vi "Append Image to Report (path).vi"(0 "report in":refnum<class "ooWriter.lvclass">, 1 "alignment (default)":T1, 2 "MS Office parameters":T2, 7 "path or URL of image":path, 9 "caption or alternative string":string, 11 "error in (no error)":errorcluster) -> (4 "report out":refnum<class "ooWriter.lvclass">, 8 "start out (Word)":i32, 10 "end out (Word)":i32, 15 "error out":errorcluster)   [LabVIEW 2009, in "ooWriter.lvclass"]
doc: "For an HTML report, the VI embeds a link to an image into the report. For a standard report, the VI appends the image from a file. You can wire either a path to the image or a string that contains the image URL to this polymorphic VI. The data type you wire to the <B>path or URL of image</B> input determines the polymorphic instance to use."
uses:
  ooWriter.lvclass
  <vilib>/Utility/NIReport.llb/HTML Report Image Alignment.ctl
  C:/Projets/LAVAG/OpenOfficeRGT/AODL/DLLs/AODL.dll
  <vilib>/Utility/NIReport.llb/NI_ReportGenerationCore.lvlib
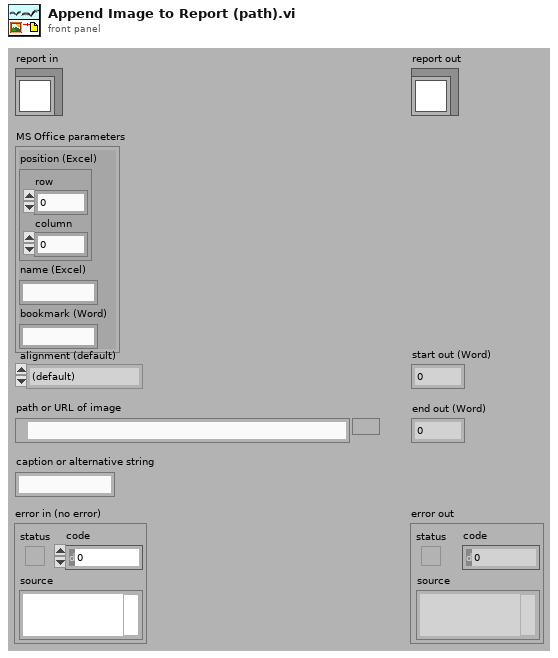
[diagram p1: front panel]
types:
  T1 = typedef "NI_ReportGenerationCore.lvlib/HTML Report Image Alignment.ctl" = enum16{"(default)", "LEFT", "RIGHT", "TOP", "TEXTTOP", "MIDDLE", "ABSMIDDLE", "BASELINE", "BOTTOM", "ABSBOTTOM"}
  T2 = cluster{"position (Excel)":cluster{"row":i32, "column":i32}, "name (Excel)":string, "bookmark (Word)":string}
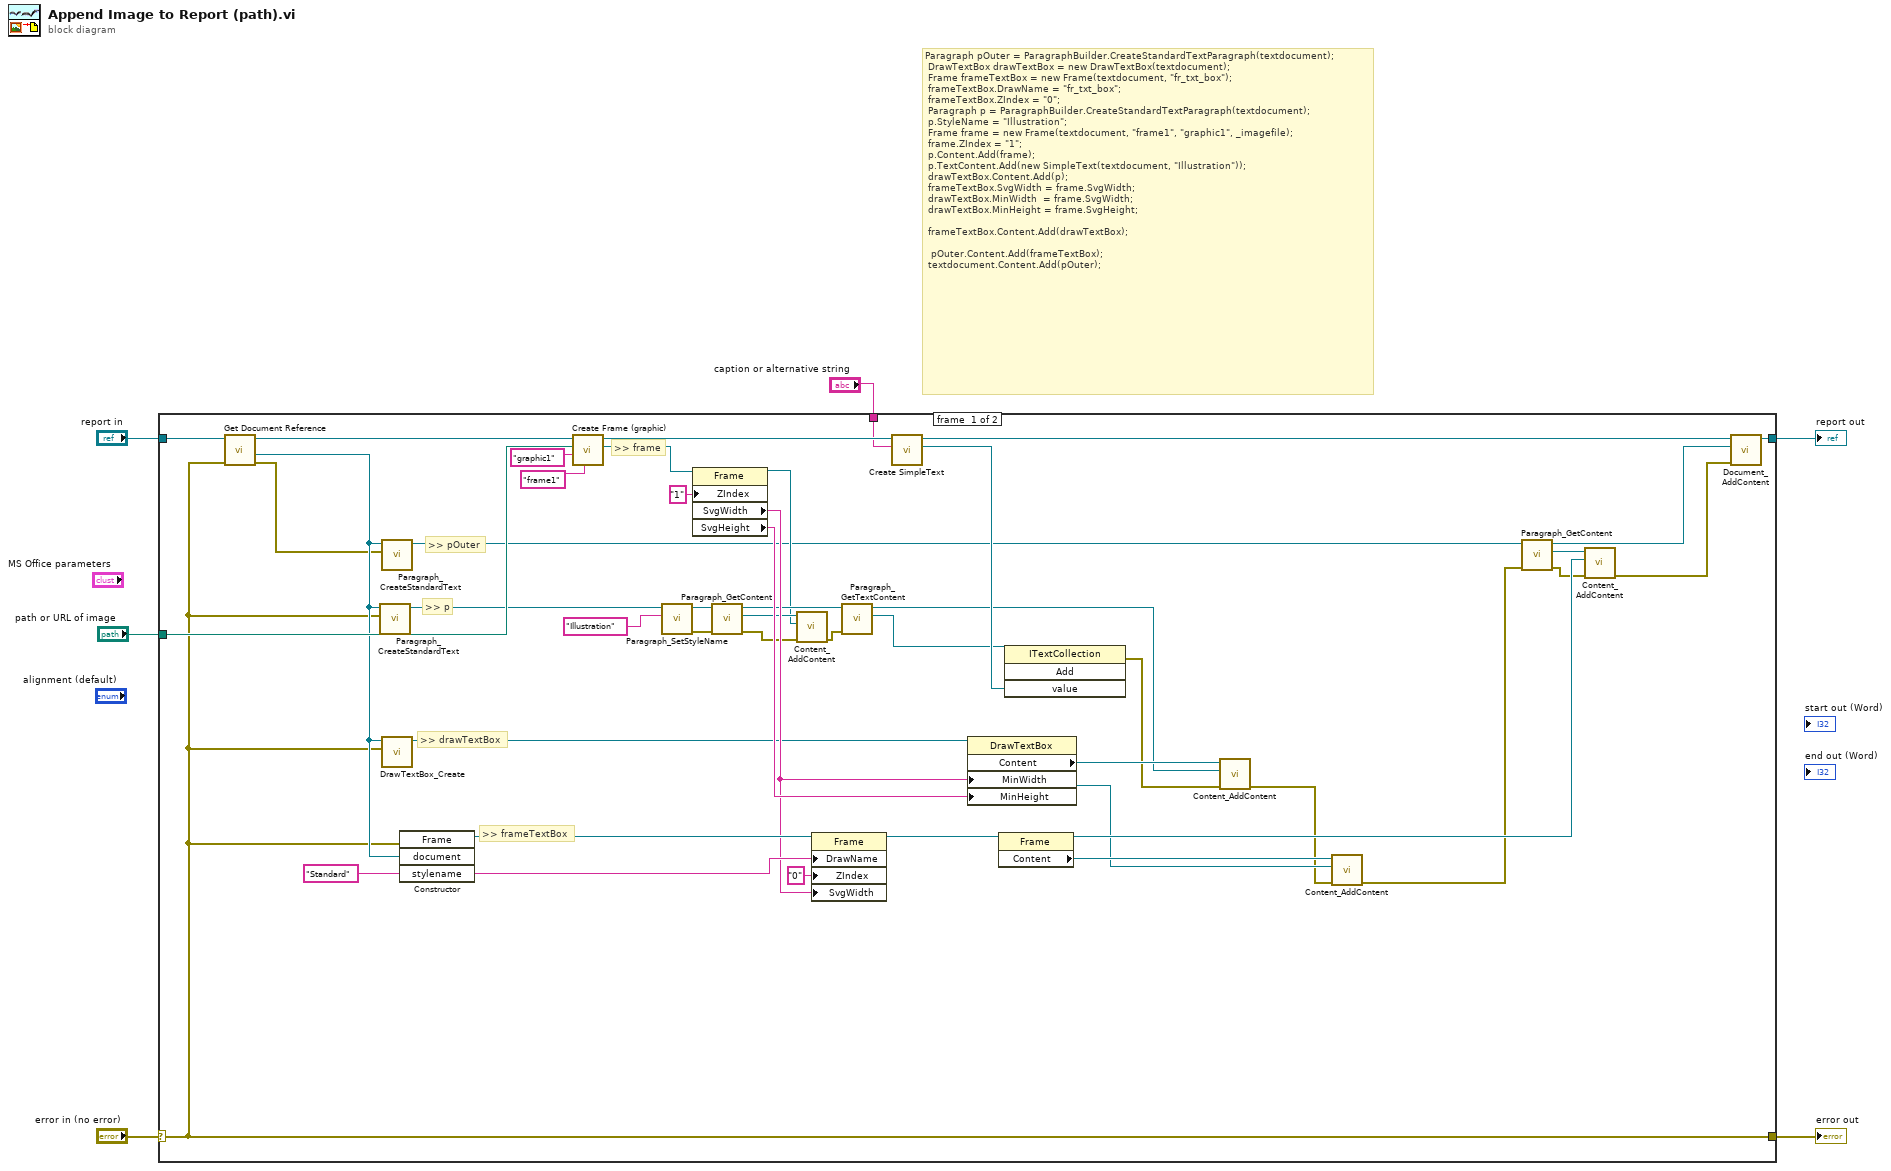
[diagram p0: block diagram]
diagram:
  # "Paragraph pOuter = ParagraphBuilder.CreateStandardTextParagraph(textdocument);\n DrawTextBox drawTextBox = new DrawTextBox(textdocument);\n Frame frameTextBox = new Frame(textdocument, \"fr_txt_box\");\n frameTextBox.DrawName = \"fr_txt_box\";\n frameTextBox.ZIndex = \"0\";\n Paragraph p = ParagraphBuilder.CreateStandardTextParagraph(textdocument);\n p.StyleName = \"Illustration\";\n Frame frame = new Frame(textdocument, \"frame1\", \"graphic1\", _imagefile);\n frame.ZIndex = \"1\";\n p.Content.Add(frame);\n p.TextContent.Add(new SimpleText(textdocument, \"Illustration\"));\n drawTextBox.Content.Add(p);\n frameTextBox.SvgWidth = frame.SvgWidth;\n drawTextBox.MinWidth  = frame.SvgWidth;\n drawTextBox.MinHeight = frame.SvgHeight;\n\n frameTextBox.Content.Add(drawTextBox);\n\n  pOuter.Content.Add(frameTextBox);\n textdocument.Content.Add(pOuter);"
  n1 = case shown="No Error" "error in (no error)" {
    selector: "error in (no error)" -> [w8 w52]
    tunnel: [w8 w52] -> w5
    tunnel: "report in" -> [w10 w53]
    tunnel: [w51 w53] -> w3
    tunnel: "path or URL of image" -> [w46 _]
    tunnel: "caption or alternative string" -> [w36 _]
    frame #0 {
      w49 = "Standard" ("frameStyleName")
      # ">> frame"
      # ">> p"
      # ">> frameTextBox"
      # ">> drawTextBox"
      # ">> pOuter"
      n2 = call-dynamic "Get Document Reference.vi"("error in (no error)"=w8, "ooDocument in"=w10) -> ("error out"=w7:errorcluster, "Document"=w11:refnum<k24>, "ooDocument out"=w9:refnum<class "ooWriter.lvclass">)  [unwired: 7 in]
      n3 = call "Paragraph_CreateStandardText.vi"("error in"=w8, "document"=w11) -> ("StandardTextParagraph"=w18:refnum<k24>)  [unwired: 8 in, 1 out]
      n4 = call "Paragraph_CreateStandardText.vi"("error in"=w7, "document"=w11) -> ("StandardTextParagraph"=w17:refnum<k24>)  [unwired: 8 in, 1 out]
      n5 = call "DrawTextBox_Create.vi"("error in"=w8, "document"=w11) -> ("DrawTextBox"=w12:refnum<k24>)  [unwired: 8 in, 1 out]
      n6 = constructor class="Frame"(error in=w8, "document"=w11, "stylename"=w49) -> (reference out=w50:refnum<k24>)  [unwired: 2 in, 4 out]
      n7 = call-dynamic "Create Frame (graphic).vi"("stylename"="frame1", "drawName"="graphic1", "Graphic file"=w46, "ooWriter in"=w9) -> ("Frame (graphic)"=w42:refnum<k24>, "ooWriter out"=w39:refnum<class "ooWriter.lvclass">)  [unwired: 5 in, 1 out]
      n8 = call "Paragraph_SetStyleName.vi"("StyleName"="Illustration", "Paragraph"=w18) -> ("error out"=w29:errorcluster, "Paragraph dup"=w33:refnum<k24>)  [unwired: 8 in]
      n9 = property class="Frame"(reference=w42, "ZIndex"="1") -> (reference out=w30:refnum<k24>, "SvgWidth"=w40:string, "SvgHeight"=w41:string)  [unwired: 1 in, 1 out]
      n10 = call "Paragraph_GetContent.vi"("error in"=w29, "Paragraph"=w33) -> ("error out"=w27:errorcluster, "ContentCollection"=w31:refnum<k24>, "Paragraph dup"=w35:refnum<k24>)  [unwired: 7 in]
      n11 = call "Content_AddContent.vi"("error in"=w27, "Content"=w30, "ContentCollection"=w31) -> ("error out"=w28:errorcluster)  [unwired: 7 in, 1 out]
      n12 = property class="Frame"(reference=w50, "DrawName"=w49, "ZIndex"="0", "SvgWidth"=w40) -> (reference out=w47:refnum<k24>)  [unwired: 1 in, 1 out]
      n13 = call "Paragraph_GetTextContent.vi"("error in"=w28, "Paragraph"=w35) -> ("TextContent Collection"=w34:refnum<k24>, "Paragraph dup"=w22:refnum<k24>)  [unwired: 7 in, 1 out]
      n14 = call-dynamic "Create SimpleText.vi"("simpleText"=w36, "ooDocument"=w39) -> ("SimpleText"=w37:refnum<k24>, "ooDocument out"=w38:refnum<class "ooWriter.lvclass">)  [unwired: 7 in, 1 out]
      n15 = property class="DrawTextBox"(reference=w12, "MinWidth"=w40, "MinHeight"=w41) -> (reference out=w20:refnum<k24>, "Content"=w24:refnum<k24>)  [unwired: 1 in, 1 out]
      n16 = property class="Frame"(reference=w47) -> (reference out=w26:refnum<k24>, "Content"=w21:refnum<k24>)  [unwired: 1 in, 1 out]
      n17 = invoke class="ITextCollection" method="Add"(reference=w34, "value"=w37) -> (error out=w23:errorcluster)  [unwired: 2 in, 3 out]
      n18 = call "Content_AddContent.vi"("error in"=w23, "Content"=w22, "ContentCollection"=w24) -> ("error out"=w19:errorcluster)  [unwired: 7 in, 1 out]
      n19 = call "Content_AddContent.vi"("error in"=w19, "Content"=w20, "ContentCollection"=w21) -> ("error out"=w13:errorcluster)  [unwired: 7 in, 1 out]
      n20 = call "Paragraph_GetContent.vi"("error in"=w13, "Paragraph"=w17) -> ("error out"=w14:errorcluster, "ContentCollection"=w15:refnum<k24>, "Paragraph dup"=w16:refnum<k24>)  [unwired: 7 in]
      n21 = call "Content_AddContent.vi"("error in"=w14, "Content"=w26, "ContentCollection"=w15) -> ("error out"=w25:errorcluster)  [unwired: 7 in, 1 out]
      n22 = call-dynamic "Document_AddContent.vi"("error in (no error)"=w25, "Content"=w16, "ooWriter in"=w38) -> ("ooWriter out"=w51:refnum<class "ooWriter.lvclass">)  [unwired: 7 in, 1 out]
    }
    frame #1 {
    }
  }
  "error out" <- w5
  "report out" <- w3
